vi "PicoScope6000GetRapidBlock.vi"(0 "error in":errorcluster, 7 "handle in":i16, 11 "Rapid Block Acquisition Settings":T1) -> (2 "Channel A Buffer":i16[][](array[numeric]), 3 "Channel B Buffer":i16[][](array[numeric]), 4 "error out":errorcluster, 6 "handle out":i16, 10 "noOfSamples":u32[](array[numeric]), 13 "Channel C Buffer":i16[][](array[numeric]), 14 "Channel D Buffer":i16[][](array[numeric]))   [LabVIEW 2009]
doc: "This VI gets a set of blocks captured using rapid block mode. It outputs two-dimensional arrays for each channel that contain data from all the requested captures."
uses:
  ps6000.dll
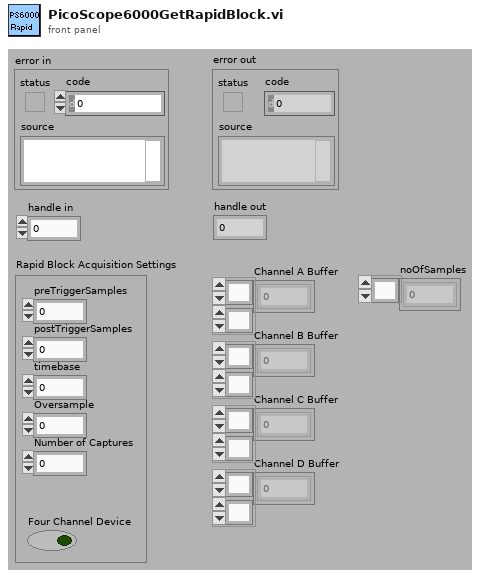
[diagram p1: front panel]
types:
  T1 = cluster{"preTriggerSamples":u32, "postTriggerSamples":u32, "timebase":u32, "Four Channel Device":bool, "Oversample":i16, "Number of Captures":u32}
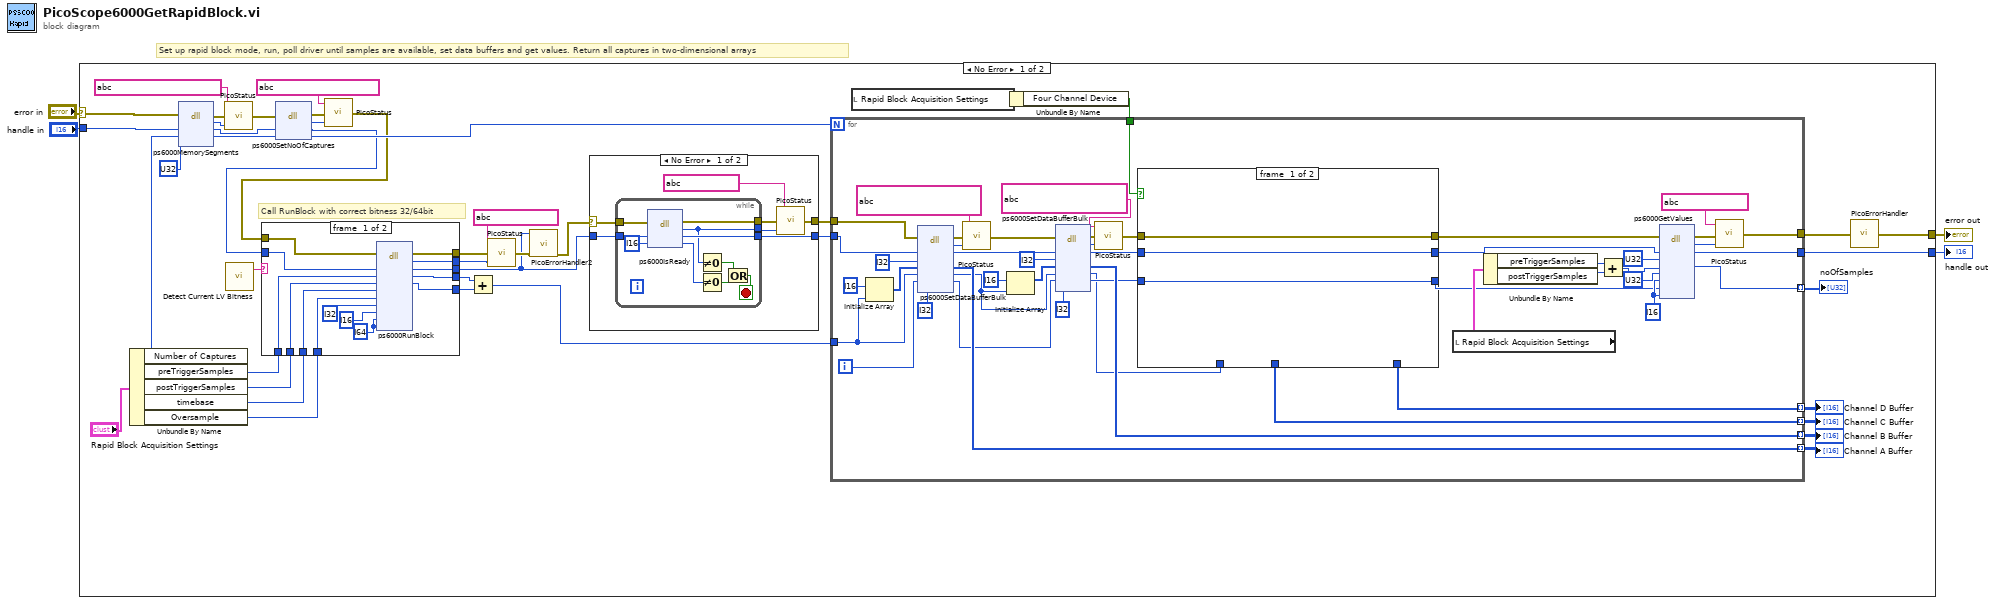
[diagram p0: block diagram]
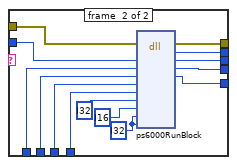
[diagram p2: hidden frame]
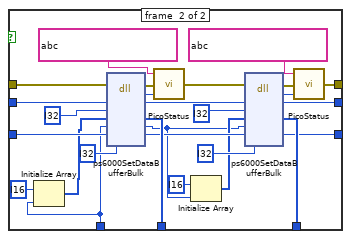
[diagram p3: hidden frame]
diagram:
  # "Set up rapid block mode, run, poll driver until samples are available, set data buffers and get values. Return all captures in two-dimensional arrays"
  n1 = case shown="No Error" "error in" {
    selector: "error in" -> [w43 w173]
    tunnel: [w22 w173] -> w3
    tunnel: "handle in" -> [w42 w172]
    tunnel: [w24 w172] -> w1
    frame #0 {
      # "Call RunBlock with correct bitness 32/64bit"
      n2 = Unbundle By Name("Rapid Block Acquisition Settings") -> ("Number of Captures"=w38:u32, "preTriggerSamples"=w10:u32, "postTriggerSamples"=w9:u32, "timebase"=w8:u32, "Oversample"=w7:i16)
      n3 = dll-call lib="PS6000.dll" fn="ps6000MemorySegments" ("ps3000.dll:_ps3000_open_unit@0")(error in=w43, "handle"=w42, "nSegments"=w38, "nMaxSamples"=u32 ?) -> (error out=w40:errorcluster, "PICO_STATUS"=w41:i32, "handle"=w35:i16, "nSegments"=w36:u32)  [unwired: 3 in, 1 out]
      n4 = call "PicoStatus.vi"("PICO STATUS"=w41, "error in"=w40, "source"=string ?) -> ("error out"=w34:errorcluster)
      n5 = call "Detect Current LV Bitness.vi"() -> ("bitness"=w17:string)  [unwired: 11 in]
      n6 = dll-call lib="PS6000.dll" fn="ps6000SetNoOfCaptures" ("ps3000.dll:_ps3000_open_unit@0")(error in=w34, "handle"=w35, "nCaptures"=w36) -> (error out=w32:errorcluster, "PICO_STATUS"=w33:i32, "handle"=w13:i16, "nCaptures"=w29:u32)  [unwired: 2 in, 1 out]
      n7 = call "PicoStatus.vi"("PICO STATUS"=w33, "error in"=w32, "source"=string ?) -> ("error out"=w14:errorcluster)
      n8 = case shown="\"32\", Default" w17 {
        tunnel: w8 -> [w61 w75]
        tunnel: w10 -> [w60 w74]
        tunnel: w9 -> [w59 w73]
        tunnel: [w58 w72] -> w21
        tunnel: [w57 w71] -> w20
        tunnel: w14 -> [w56 w70]
        tunnel: w13 -> [w55 w69]
        tunnel: w7 -> [w54 w68]
        tunnel: [w53 w67] -> w11
        tunnel: [w49 w63] -> w16
        tunnel: [w48 w62] -> w15
        frame #0 {
          w51 = i64 ? ("pParameter")
          n9 = dll-call lib="PS6000.dll" fn="ps6000RunBlock" ("ps3000.dll:_ps3000_open_unit@0")(error in=w56, "handle"=w55, "preTriggerSamples"=w60, "postTriggerSamples"=w59, "timebase"=w61, "oversample"=w54, "timeindisposed"=i32 ? ("pParameter"), "segmentIndex"=i16 ? ("pParameter"), "lpReady"=w51, "pParameter"=w51) -> (error out=w57:errorcluster, "PICO_STATUS"=w58:u32, "handle"=w53:i16, "preTriggerSamples"=w48:u32, "postTriggerSamples"=w49:u32)  [unwired: 8 in, 1 out]
        }
        frame #1 {
          w65 = i32 ? ("pParameter")
          n10 = dll-call lib="PS6000.dll" fn="ps6000RunBlock" ("ps3000.dll:_ps3000_open_unit@0")(error in=w70, "handle"=w69, "preTriggerSamples"=w74, "postTriggerSamples"=w73, "timebase"=w75, "oversample"=w68, "timeindisposed"=i32 ? ("pParameter"), "segmentIndex"=i16 ? ("pParameter"), "lpReady"=w65, "pParameter"=w65) -> (error out=w71:errorcluster, "PICO_STATUS"=w72:u32, "handle"=w67:i16, "preTriggerSamples"=w62:u32, "postTriggerSamples"=w63:u32)  [unwired: 8 in, 1 out]
        }
      }
      n11 = Add(x=w15, y=w16) -> (x+y=w6:u32)
      n12 = call "PicoStatus.vi"("PICO STATUS"=w21, "error in"=w20, "source"=string ?) -> ("error out"=w18:errorcluster)
      n13 = call "PicoErrorHandler2.vi"("error in (no error)"=w18, "handle In"=w11) -> ("error out"=w12:errorcluster)  [unwired: 9 in]
      n14 = case shown="No Error" w12 {
        selector: w12 -> [w157 w170]
        tunnel: w11 -> [w159 w171]
        tunnel: [w158 w171] -> w47
        tunnel: [w156 w170] -> w46
        frame #0 {
          n15 = while {
            tunnel: [w169] -> w158
            tunnel: w159 -> [w168]
            tunnel: [w163] -> w154
            tunnel: w157 -> [w162]
            tunnel: [w161] -> w155
            stop <- w167 stop-if-true
            n16 = dll-call lib="PS6000.dll" fn="ps6000IsReady" ("ps3000.dll:_ps3000_open_unit@0")(error in=w162, "handle"=w168, "ready"=i16 ?) -> (error out=w161:errorcluster, "status"=w163:i32, "handle"=w169:i16, "ready"=w164:i16)  [unwired: 2 in, 1 out]
            n17 = Not Equal To 0?(x=w163) -> (x != 0?=w165:bool)
            n18 = Not Equal To 0?(x=w164) -> (x != 0?=w166:bool)
            n19 = Or(x=w165, y=w166) -> (x .or. y?=w167:bool)
          }
          n20 = call "PicoStatus.vi"("PICO STATUS"=w154, "error in"=w155, "source"=string ?) -> ("error out"=w156:errorcluster)
        }
        frame #1 {
        }
      }
      n21 = local read "Rapid Block Acquisition Settings"() -> (w30:T1)
      n22 = Unbundle By Name(w30) -> ("Four Channel Device"=w44:bool)
      n23 = for {
        N: w29 -> [_]
        tunnel: w47 -> [w122]
        tunnel: w46 -> [w117]
        tunnel: w44 -> [w108]
        tunnel: [w111] -> w28 mode=indexing
        tunnel: [w110] -> w27 mode=indexing
        tunnel: [w84] -> w26 mode=indexing
        tunnel: [w106] -> w25 mode=indexing
        tunnel: w6 -> [w109]
        tunnel: [w93] -> w24
        tunnel: [w79] -> w23
        tunnel: [w76] -> w5 mode=indexing
        i -> [w107]
        w105 = i16 ? ("overflow")
        n24 = Initialize Array(i16 ? ("element"), w109) -> (w121:i16[])
        n25 = dll-call lib="PS6000.dll" fn="ps6000SetDataBufferBulk" ("ps3000.dll:_ps3000_open_unit@0")(error in=w117, "handle"=w122, "channel"=i32 ?, "buffer"=w121, "bufferLth"=w109, "waveform"=w107, "downSampleRatioMode"=i32 ?) -> (error out=w115:errorcluster, "PICO_STATUS"=w116:i32, "handle"=w89:i16, "buffer"=w106:i16[], "bufferLth"=w86:u32, "waveform"=w85:u32)  [unwired: 4 in, 1 out]
        n26 = call "PicoStatus.vi"("PICO STATUS"=w116, "error in"=w115, "source"=string ?) -> ("error out"=w90:errorcluster)
        n27 = Initialize Array(i16 ? ("element"), w86) -> (w87:i16[])
        n28 = dll-call lib="PS6000.dll" fn="ps6000SetDataBufferBulk" ("ps3000.dll:_ps3000_open_unit@0")(error in=w90, "handle"=w89, "channel"=i32 ?, "buffer"=w87, "bufferLth"=w86, "waveform"=w85, "downSampleRatioMode"=i32 ?) -> (error out=w92:errorcluster, "PICO_STATUS"=w91:i32, "handle"=w83:i16, "buffer"=w84:i16[], "bufferLth"=w77:u32, "waveform"=w82:u32)  [unwired: 4 in, 1 out]
        n29 = call "PicoStatus.vi"("PICO STATUS"=w91, "error in"=w92, "source"=string ?) -> ("error out"=w114:errorcluster)
        n30 = case shown="True" w108 {
          tunnel: w83 -> [w125 w144]
          tunnel: [w125 w138] -> w95
          tunnel: [_ w140] -> w111
          tunnel: [_ w147] -> w110
          tunnel: w114 -> [w124 w143]
          tunnel: [w124 w152] -> w96
          tunnel: w77 -> [_ w127]
          tunnel: w82 -> [w123 w146]
          tunnel: [w123 w139] -> w94
          frame #0 {
          }
          frame #1 {
            n31 = Initialize Array(i16 ? ("element"), w127) -> (w130:i16[])
            n32 = dll-call lib="PS6000.dll" fn="ps6000SetDataBufferBulk" ("ps3000.dll:_ps3000_open_unit@0")(error in=w143, "handle"=w144, "channel"=i32 ?, "buffer"=w130, "bufferLth"=w127, "waveform"=w146, "downSampleRatioMode"=i32 ?) -> (error out=w149:errorcluster, "PICO_STATUS"=w148:i32, "handle"=w137:i16, "buffer"=w147:i16[], "bufferLth"=w126:u32, "waveform"=w134:u32)  [unwired: 4 in, 1 out]
            n33 = call "PicoStatus.vi"("PICO STATUS"=w148, "error in"=w149, "source"=string ?) -> ("error out"=w136:errorcluster)
            n34 = Initialize Array(i16 ? ("element"), w126) -> (w128:i16[])
            n35 = dll-call lib="PS6000.dll" fn="ps6000SetDataBufferBulk" ("ps3000.dll:_ps3000_open_unit@0")(error in=w136, "handle"=w137, "channel"=i32 ?, "buffer"=w128, "bufferLth"=w126, "waveform"=w134, "downSampleRatioMode"=i32 ?) -> (error out=w142:errorcluster, "PICO_STATUS"=w141:i32, "handle"=w138:i16, "buffer"=w140:i16[], "waveform"=w139:u32)  [unwired: 5 in, 1 out]
            n36 = call "PicoStatus.vi"("PICO STATUS"=w141, "error in"=w142, "source"=string ?) -> ("error out"=w152:errorcluster)
          }
        }
        n37 = local read "Rapid Block Acquisition Settings"() -> (w101:T1)
        n38 = Unbundle By Name(w101) -> ("preTriggerSamples"=w103:u32, "postTriggerSamples"=w102:u32)
        n39 = Add(x=w103, y=w102) -> (x+y=w104:u32)
        n40 = dll-call lib="PS6000.dll" fn="ps6000GetValues" ("ps3000.dll:_ps3000_open_unit@0")(error in=w96, "handle"=w95, "startIndex"=u32 ?, "noOfSamples"=w104, "downSampleRatio"=u32 ?, "downSampleRatioMode"=w105, "segmentIndex"=w94, "overflow"=w105) -> (error out=w98:errorcluster, "PICO_STATUS"=w97:i32, "handle"=w93:i16, "noOfSamples"=w76:u32)  [unwired: 7 in, 1 out]
        n41 = call "PicoStatus.vi"("PICO STATUS"=w97, "error in"=w98, "source"=string ?) -> ("error out"=w79:errorcluster)
      }
      "Channel D Buffer" <- w28
      "Channel C Buffer" <- w27
      "Channel B Buffer" <- w26
      "Channel A Buffer" <- w25
      "noOfSamples" <- w5
      n42 = call "PicoErrorHandler.vi"("error in"=w23) -> ("error out"=w22:errorcluster)
    }
    frame #1 {
    }
  }
  "error out" <- w3
  "handle out" <- w1
